vi "TMS Robot.vi"() -> ()   [LabVIEW 2018]
uses:
  <vilib>/Platform/TimedLoop/XDataNode/timing_clust.ctl
  <vilib>/Platform/TimedLoop/XDataNode/nitl_modes.ctl
  <vilib>/Platform/TimedLoop/XDataNode/wakeup.ctl
  <vilib>/myRIO/Instrument Drivers/Onboard IO/AI/typedefs/AI Reference.ctl
  <vilib>/myRIO/Common/Instrument Driver Framework/Utilities/typedefs/myRIO Generic Hardware Reference.ctl
  <vilib>/myRIO/Common/Instrument Driver Framework/Utilities/typedefs/Hardware Version Enum.ctl
  <vilib>/myRIO/Common/Instrument Driver Framework/Utilities/typedefs/myRIO v1.0 Reference.ctl
  <vilib>/myRIO/Common/Instrument Driver Framework/Utilities/typedefs/Generic FPGA Reference.ctl
  <vilib>/myRIO/Common/Instrument Driver Framework/myRIO v1.0/AI/typedefs/AI Channels List.ctl
  <vilib>/myRIO/Common/Instrument Driver Framework/myRIO v1.0/AI/typedefs/AI Channels Enum.ctl
  <vilib>/myRIO/Common/Instrument Driver Framework/Utilities/typedefs/Analog Scaling Constants List.ctl
  <vilib>/myRIO/Common/Instrument Driver Framework/Utilities/typedefs/Analog Scaling Constants.ctl
  <vilib>/userdefined/High Color/nirio_resource_hc.ctl
  <vilib>/myRIO/Instrument Drivers/Onboard IO/DIO/typedefs/DIO Reference.ctl
  <vilib>/myRIO/Common/Instrument Driver Framework/myRIO v1.0/DIO/typedefs/DIO Channels List.ctl
  <vilib>/myRIO/Common/Instrument Driver Framework/myRIO v1.0/DIO/typedefs/DIO Channels Enum.ctl
  <vilib>/myRIO/Common/Instrument Driver Framework/myRIO v1.0/AI/vis/myRIO v1.1 Open AI.vi
  <vilib>/myRIO/Common/Instrument Driver Framework/myRIO v1.0/DIO/vis/myRIO v1.1 Open DIO.vi
  <vilib>/myRIO/Common/Instrument Driver Framework/Utilities/vis/Validate Channels.vi
  <vilib>/myRIO/Common/Instrument Driver Framework/myRIO v1.0/AI/vis/myRIO v1.0 Reserve AI.vi
  <vilib>/myRIO/Common/Instrument Driver Framework/myRIO v1.0/DIO/vis/myRIO v1.0 Reserve DIO.vi
  <vilib>/myRIO/Common/Instrument Driver Framework/myRIO v1.0/DIO/vis/myRIO v1.0 Close DIO.vi
  <vilib>/myRIO/Common/Instrument Driver Framework/myRIO v1.0/AI/vis/myRIO v1.0 Build MUX Configuration AI.vi
  <vilib>/myRIO/Common/Instrument Driver Framework/myRIO v1.0/Resource Manager/vis/myRIO v1.0 Reserve Channel List.vi
  <vilib>/myRIO/Common/Instrument Driver Framework/myRIO v1.0/DIO/vis/myRIO v1.0 Build MUX Configuration DIO.vi
  <vilib>/myRIO/Common/Instrument Driver Framework/myRIO v1.0/DIO/vis/myRIO v1.0 Unreserve DIO.vi
  <vilib>/myRIO/Common/Instrument Driver Framework/myRIO v1.0/Resource Manager/vis/myRIO v1.0 Reserve Channel.vi
  <vilib>/myRIO/Common/Instrument Driver Framework/myRIO v1.0/Resource Manager/vis/myRIO v1.0 Unreserve Channel.vi
  <vilib>/myRIO/Common/Instrument Driver Framework/myRIO v1.0/Resource Manager/vis/myRIO v1.0 Create Configuration List.vi
  <vilib>/myRIO/Common/Instrument Driver Framework/myRIO v1.0/Resource Manager/vis/myRIO v1.0 Unreserve Channel List.vi
  <vilib>/myRIO/Common/Instrument Driver Framework/myRIO v1.0/Resource Manager/vis/myRIO v1.0 Build Mutex Name.vi
  <vilib>/Utility/VariantDataType/GetNumericInfo.vi
  <vilib>/Utility/error.llb/Error Cluster From Error Code.vi
  <vilib>/myRIO/Common/Instrument Driver Framework/myRIO v1.0/myRIO v1.1 Open.vi
  <vilib>/myRIO/Common/Instrument Driver Framework/Utilities/vis/IO Manager.vi
  <vilib>/myRIO/Common/Instrument Driver Framework/Utilities/vis/Configuration Manager.vi
  <vilib>/myRIO/Common/Instrument Driver Framework/myRIO v1.0/Resource Manager/vis/myRIO v1.0 Configure IO.vi
  <vilib>/myRIO/Common/Instrument Driver Framework/myRIO v1.0/myRIO v1.0 Close.vi
  <vilib>/myRIO/Common/Instrument Driver Framework/myRIO v1.0/AI/vis/myRIO v1.0 Get Scaling Constants AI.vi
  <vilib>/myRIO/Common/Instrument Driver Framework/myRIO v1.0/AI/vis/myRIO v1.0 Read AI.vi
  <vilib>/myRIO/Common/Instrument Driver Framework/myRIO v1.0/DIO/vis/myRIO v1.0 Write DIO.vi
  <vilib>/myRIO/Common/Instrument Driver Framework/myRIO v1.0/DIO/vis/myRIO v1.0 Shutdown DIO.vi
  <vilib>/platform/TimedLoop/XDataNode/XDataNode.xnode
  <vilib>/myRIO/Instrument Drivers/Onboard IO/DIO/vis/myRIO DIO Open.xnode
  <vilib>/myRIO/Instrument Drivers/Onboard IO/AI/vis/myRIO AI Open.xnode
  <vilib>/Platform/TimedLoop/XDataNode/XDNodeRunTimeDep.lvlib
  <vilib>/myRIO/Instrument Drivers/Onboard IO/DIO/DIO.lvlib
  <vilib>/myRIO/Instrument Drivers/Onboard IO/AI/AI.lvlib
panel:
  in  "Stop number L":dbl
  in  "Stop number R":dbl
  in  "Stop number x":dbl
  in  "Stop number y":dbl
  in  "Stop number z":dbl
  in  "Stop number psi":dbl
  out "up L":bool
  out "left L":bool
  in  "Step/s  curve":dbl=4.0
  in  "Step difference L":dbl
  in  "Tab Control":enum32{"Azimuth", "Elevation"}(tab)
  in  "Right":bool
  in  "Left":bool
  out "Real Output theta":dbl
  in  "User Input theta":dbl min=-45.0 max=45.0
  in  "Up":bool
  in  "Down":bool
  out "Real Output Phi":dbl
  in  "User Input Phi":dbl=10.45218049 min=9.2427 max=53.19163884
  in  "Motor Input L":dbl
  out "down L":bool
  out "right L":bool
  out "Moving":bool
  out "up R":bool
  out "left R":bool
  in  "Step difference R":dbl
  in  "Motor Input R":dbl
  out "down R":bool
  out "right R":bool
  out "Moving R":bool
  out "up z":bool
  out "down z":bool
  out "right z":bool
  out "left z":bool
  in  "Step/s z":dbl=4.0
  out "Motor Position z":dbl
  in  "User Input z":dbl min=-25.0 max=25.0
  out "Motor State z":dbl
  out "Real Output z":dbl
  in  "Step diff z":dbl
  in  "Up z":bool
  in  "Motor Input z":dbl
  in  "Down z":bool
  out "Moving z":bool
  out "up x":bool
  out "down x":bool
  out "right x":bool
  out "left x":bool
  in  "Step/s x":dbl=4.0
  out "Motor Position x":dbl
  in  "User Input x":dbl min=-25.0 max=25.0
  out "Motor State x":dbl
  out "Real Output x":dbl
  in  "Step diff x":dbl
  in  "Forward x":bool
  in  "Motor Input x":dbl
  in  "Backward x":bool
  out "Moving x":bool
  out "up y":bool
  out "down y":bool
  out "right y":bool
  out "left y":bool
  in  "Step/s y":dbl=4.0
  out "Motor Position y":dbl
  in  "User Input y":dbl min=-25.0 max=25.0
  out "Motor State y":dbl
  out "Real Output y":dbl
  in  "Step diff y":dbl
  in  "Left y":bool
  in  "Motor Input y":dbl
  in  "Right y":bool
  out "Moving y":bool
  out "up psi":bool
  out "down psi":bool
  out "right psi":bool
  out "left psi":bool
  in  "Step/s psi":dbl=4.0
  out "Motor Position psi":dbl
  in  "User Input psi":dbl min=-90.0 max=90.0
  out "Motor State psi":dbl
  out "Real Output psi":dbl
  in  "Step diff psi":dbl
  in  "Left psi":bool
  in  "Motor Input psi":dbl
  in  "Right psi":bool
  out "Moving psi":bool
  out "Homing x":bool
  out "Homing y":bool
  out "Homing z":bool
  out "Homing":bool
  out "Homing psi":bool
  in  "Stop":bool
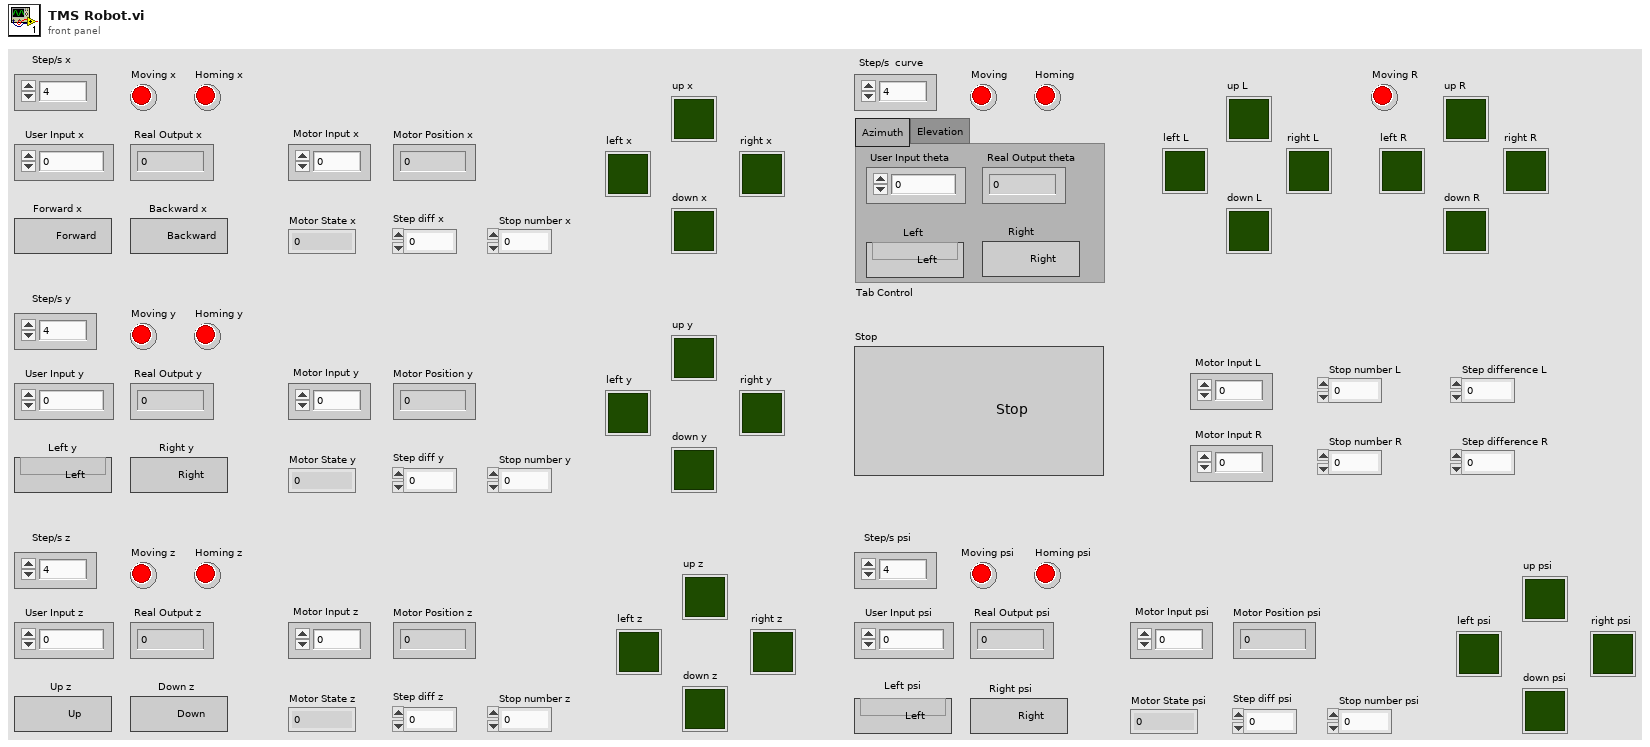
[diagram p1: front panel]
types:
  T1 = typedef "nirio_resource_hc.ctl" = tag
  T2 = typedef "Hardware Version Enum.ctl" = enum16{"Unknown", "myRIO-1900", "myRIO-1950", "roboRIO", "NI ELVIS RIO CM", "ELVIS III"}
  T3 = typedef "XDNodeRunTimeDep.lvlib/timing_clust.ctl" = cluster{"Expected End [f-1]":u64, "Actual End [f-1]":u64, "Finished Late? [f-1]":bool, "Expected End [i-1]":u64, "Actual End [i-1]":u64, "Finished Late? [i-1]":bool, "Expected Start [i]":u64, "Actual Start [i]":u64, "Expected Start [f]":u64, "Actual Start [f]":u64, "Source Name":string, "Structure Name":string, "Period":i64, "Deadline":i64, "Offset":i64, "Start":i64, "Priority":i32, "Timeout":i32, "Mode":T4, "Wakeup Reason":T5, "Error":errorcluster, "Source Type":string, "Secondary Source Type":string, "Global End Time":u64, "Global Start Time":u64, "Frame Duration":u64, "Iteration Duration":u64, "Assigned CPU":i32, "I/O Scan Engine Mode":u32}
  T4 = typedef "XDNodeRunTimeDep.lvlib/nitl_modes.ctl" = enum32{"No Change", "Process missed periods, maintain original phase", "Discard missed periods, maintain original phase", "Process missed periods, ignore original phase", "Discard missed periods, ignore original phase"}
  T5 = typedef "XDNodeRunTimeDep.lvlib/wakeup.ctl" = enum32{"Normal", "Aborted", "Asynchronous wakeup", "Timing source error", "Timed loop error", "Timeout"}
  T6 = typedef "AI.lvlib/AI Reference.ctl" = cluster{"myRIO Reference":T7, "AI Channels List":T10, "AI Scaling Constants List":T12}
  T7 = typedef "myRIO Generic Hardware Reference.ctl" = cluster{"myRIO Model":T2, "myRIO Hardware Reference":T8}
  T8 = typedef "myRIO v1.0 Reference.ctl" = cluster{"Generic FPGA Reference":T9, "Allow multiple opens":bool}
  T9 = typedef "Generic FPGA Reference.ctl" = refnum<k20>
  T10 = typedef "AI Channels List.ctl" = T11[]
  T11 = typedef "AI Channels Enum.ctl" = enum16{"Not Connected", "AudioIn/Left", "AudioIn/Right", "C/AI0", "C/AI1", "A/AI0", "A/AI1", "A/AI2", "A/AI3", "A/AI4", "A/AI5", "A/AI6", "A/AI7", "B/AI0", "B/AI1", "B/AI2", "B/AI3", "B/AI4", "B/AI5", "B/AI6", "B/AI7", "AI/AI0", "AI/AI1", "AI/AI2", "AI/AI3", "A/AI0 (DIFF)", "A/AI1 (DIFF)", "A/AI2 (DIFF)", "A/AI3 (DIFF)", "B/AI0 (DIFF)", "B/AI1 (DIFF)", "B/AI2 (DIFF)", "B/AI3 (DIFF)"}
  T12 = typedef "Analog Scaling Constants List.ctl" = T13[]
  T13 = typedef "Analog Scaling Constants.ctl" = cluster{"LSB Weight (Volts)":dbl, "Offset (Volts)":dbl, "Signed?":bool}
  T14 = typedef "DIO.lvlib/DIO Reference.ctl" = cluster{"myRIO Reference":T7, "DIO Channels List":T15}
  T15 = typedef "DIO Channels List.ctl" = T16[]
  T16 = typedef "DIO Channels Enum.ctl" = enum16{"Not Connected", "C/DIO0", "C/DIO1", "C/DIO2", "C/DIO3", "C/DIO4", "C/DIO5", "C/DIO6", "C/DIO7", "A/DIO0", "A/DIO1", "A/DIO2", "A/DIO3", "A/DIO4", "A/DIO5", "A/DIO6", "A/DIO7", "A/DIO8", "A/DIO9", "A/DIO10", "A/DIO11", "A/DIO12", "A/DIO13", "A/DIO14", "A/DIO15", "A/DIO16", "A/DIO17", "A/DIO18", "A/DIO19", "B/DIO0", "B/DIO1", "B/DIO2", "B/DIO3", "B/DIO4", "B/DIO5", "B/DIO6", "B/DIO7", "B/DIO8", "B/DIO9", "B/DIO10", "B/DIO11", "B/DIO12", "B/DIO13", "B/DIO14", "B/DIO15", "B/DIO16", "B/DIO17", "B/DIO18", "B/DIO19", "LED0", "LED1", "LED2", "LED3", "Button0", "DIO/DIO0", "DIO/DIO1", "DIO/DIO2", "DIO/DIO3", "DIO/DIO4", "DIO/DIO5", "DIO/DIO6", "DIO/DIO7", "DIO/DIO8", "DIO/DIO9", "SPI/CS0", "SPI/CS1", "SPI/CS2", "SPI/CS3", "LED RADIO (Green)", "LED RADIO (Red)", "LED COMM (Green)", "LED COMM (Red)", "LED MODE (Green)", "LED MODE (Red)"}
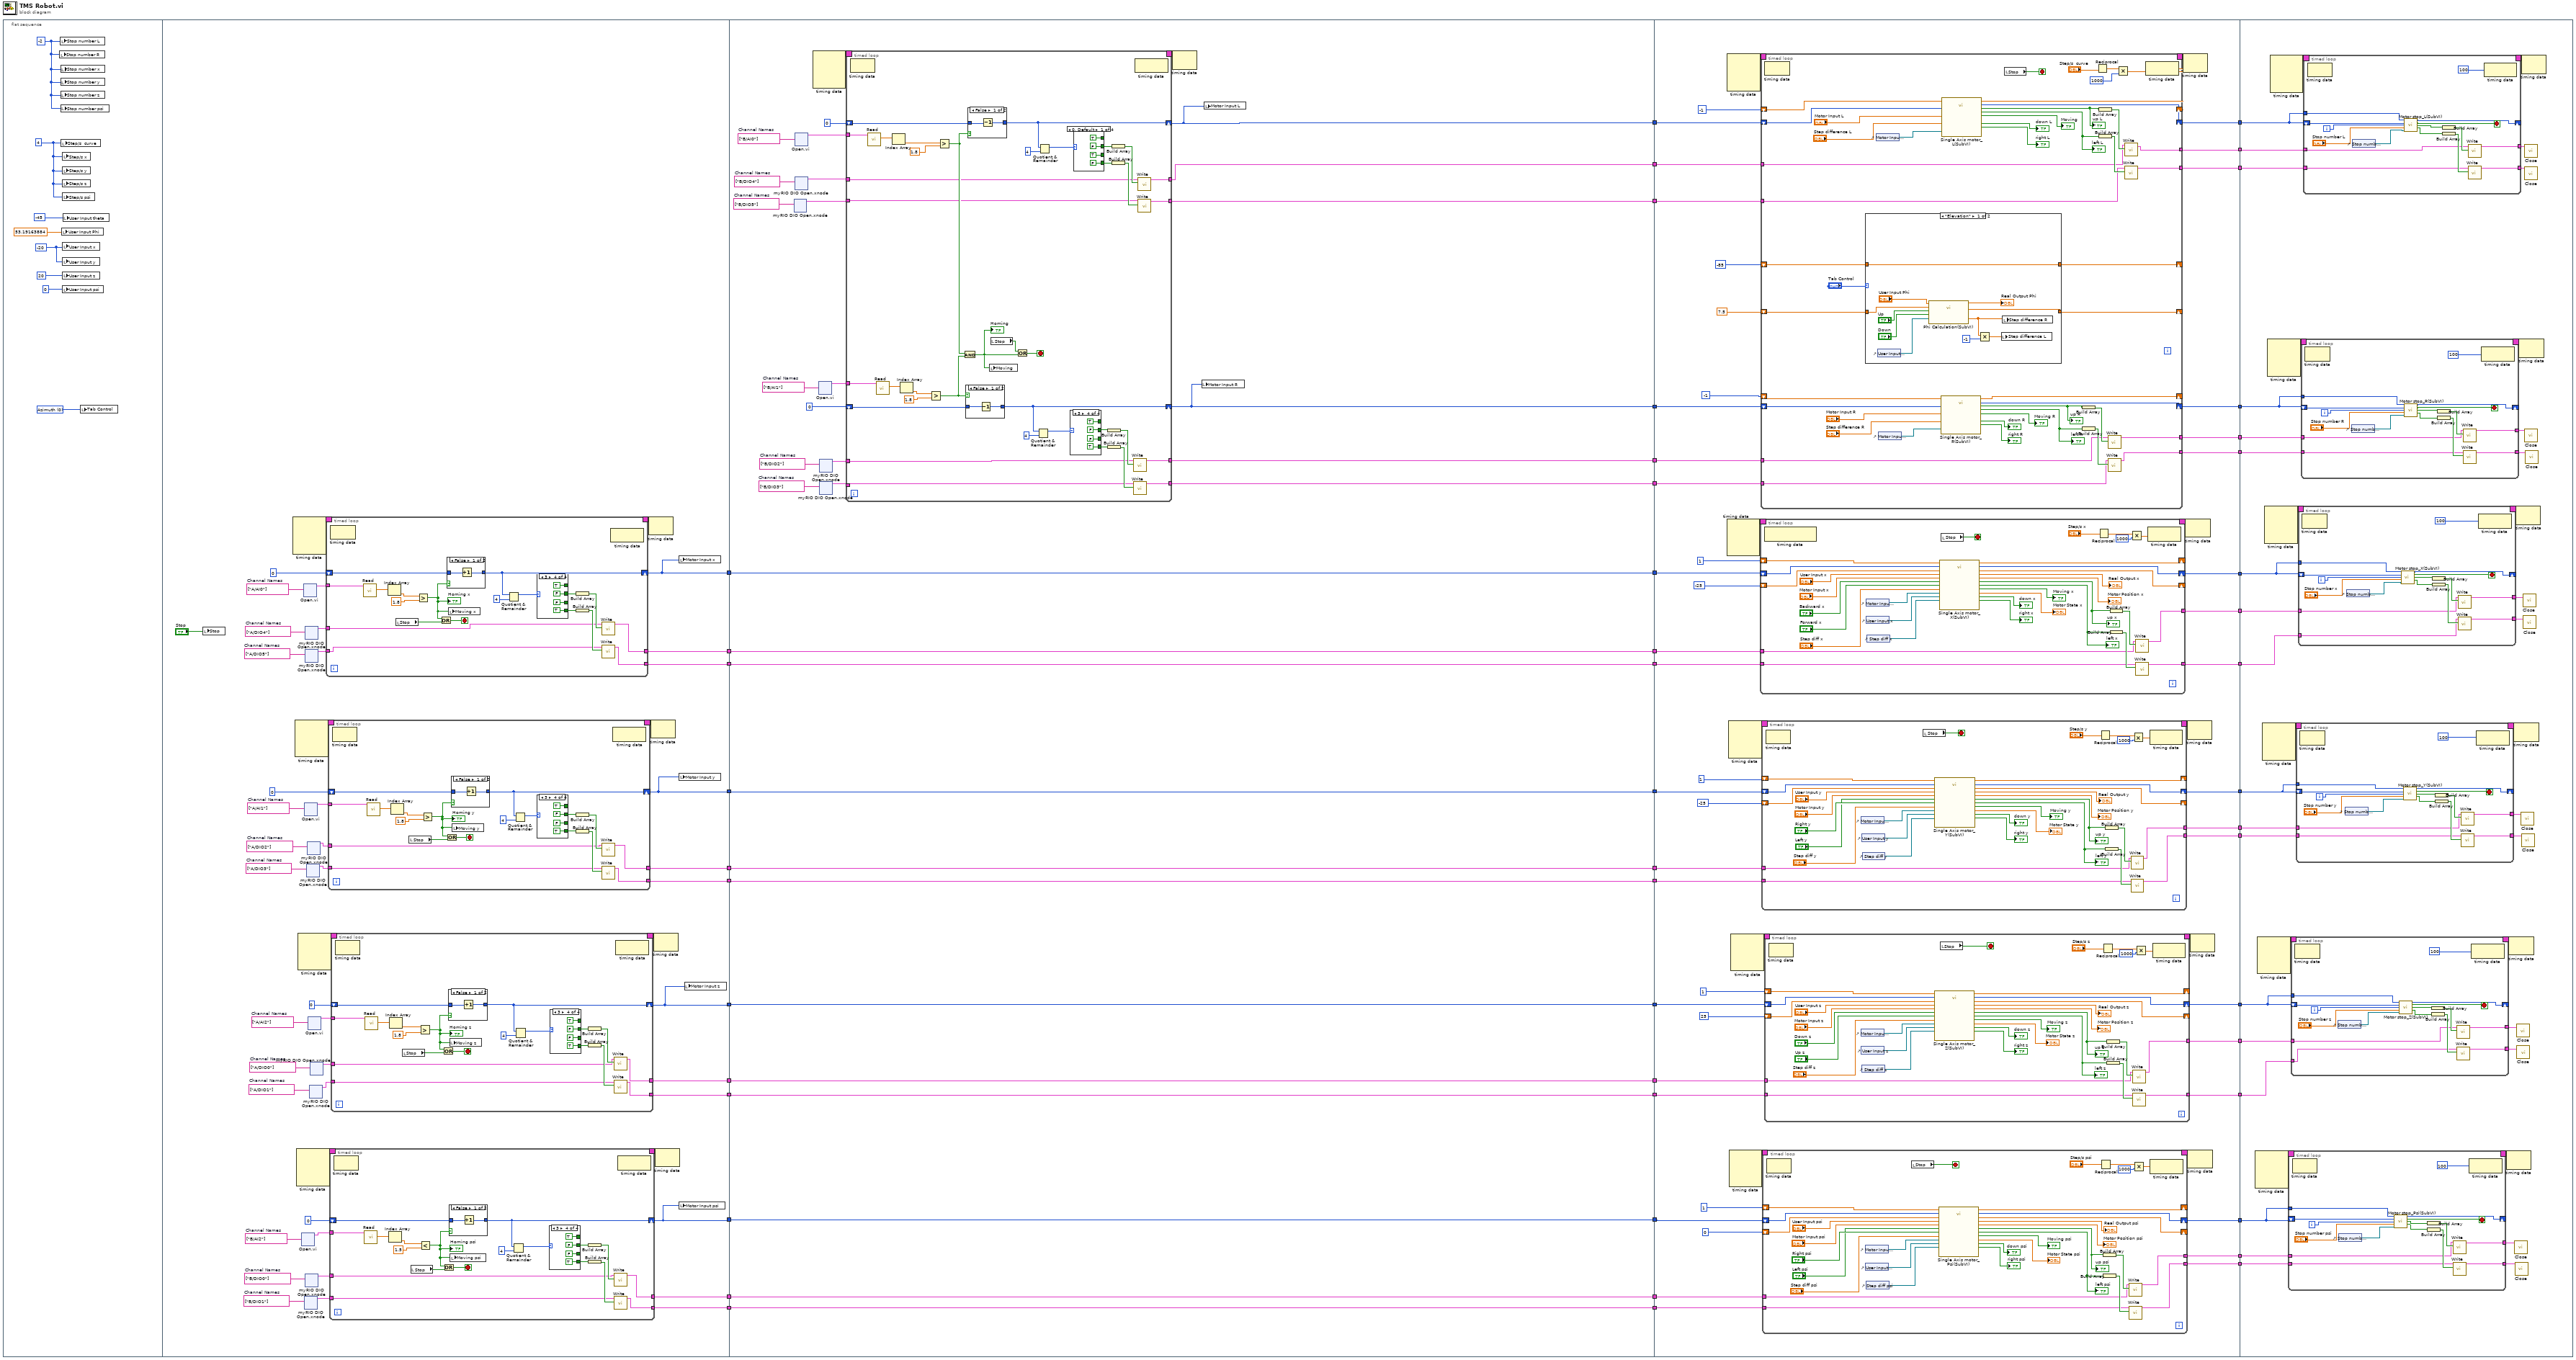
[diagram p0: block diagram]
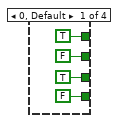
[diagram p2: hidden frame]
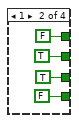
[diagram p3: hidden frame]
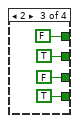
[diagram p4: hidden frame]
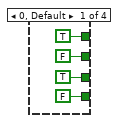
[diagram p6: hidden frame]
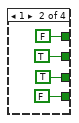
[diagram p7: hidden frame]
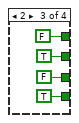
[diagram p8: hidden frame]
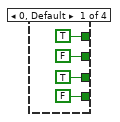
[diagram p10: hidden frame]
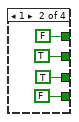
[diagram p11: hidden frame]
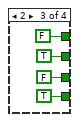
[diagram p12: hidden frame]
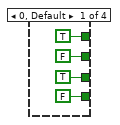
[diagram p15: hidden frame]
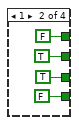
[diagram p16: hidden frame]
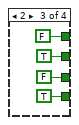
[diagram p17: hidden frame]
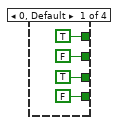
[diagram p18: hidden frame]
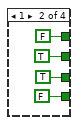
[diagram p19: hidden frame]
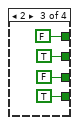
[diagram p20: hidden frame]
diagram:
  n1 = flat-sequence {
    tunnel: [w92] -> w30
    tunnel: [w91] -> w28
    tunnel: [w93] -> w26
    tunnel: [w90] -> w24
    tunnel: [w72] -> w22
    tunnel: [w71] -> w20
    tunnel: [w70] -> w18
    tunnel: [w69] -> w16
    tunnel: [w68] -> w14
    tunnel: [w67] -> w12
    tunnel: [w66] -> w10
    tunnel: [w65] -> w8
    tunnel: w30 -> [w507]
    tunnel: [w507] -> w29
    tunnel: w28 -> [w506]
    tunnel: [w506] -> w27
    tunnel: w26 -> [w505]
    tunnel: [w505] -> w25
    tunnel: w24 -> [w504]
    tunnel: [w504] -> w23
    tunnel: w22 -> [w503]
    tunnel: [w503] -> w21
    tunnel: w20 -> [w502]
    tunnel: [w502] -> w19
    tunnel: w18 -> [w501]
    tunnel: [w501] -> w17
    tunnel: w16 -> [w500]
    tunnel: [w500] -> w15
    tunnel: w14 -> [w499]
    tunnel: [w499] -> w13
    tunnel: w12 -> [w498]
    tunnel: [w498] -> w11
    tunnel: w10 -> [w497]
    tunnel: [w497] -> w9
    tunnel: w8 -> [w496]
    tunnel: [w496] -> w7
    tunnel: [w485] -> w6
    tunnel: [w484] -> w5
    tunnel: [w483] -> w4
    tunnel: [w482] -> w3
    tunnel: [w481] -> w2
    tunnel: [w480] -> w1
    tunnel: w29 -> [w723]
    tunnel: w27 -> [w722]
    tunnel: w25 -> [w721]
    tunnel: w23 -> [w719]
    tunnel: [w717] -> w48
    tunnel: [w716] -> w47
    tunnel: [w715] -> w46
    tunnel: [w714] -> w45
    tunnel: [w713] -> w44
    tunnel: [w712] -> w43
    tunnel: w21 -> [w710]
    tunnel: w19 -> [w709]
    tunnel: w17 -> [w708]
    tunnel: w15 -> [w707]
    tunnel: w13 -> [w706]
    tunnel: w11 -> [w705]
    tunnel: w9 -> [w704]
    tunnel: w7 -> [w703]
    tunnel: [w698] -> w42
    tunnel: [w697] -> w41
    tunnel: [w696] -> w40
    tunnel: [w695] -> w39
    tunnel: [w694] -> w38
    tunnel: [w693] -> w37
    tunnel: [w692] -> w36
    tunnel: [w691] -> w35
    tunnel: [w690] -> w34
    tunnel: [w689] -> w33
    tunnel: [w688] -> w32
    tunnel: [w687] -> w31
    tunnel: w6 -> [w701]
    tunnel: w5 -> [w702]
    tunnel: w4 -> [w711]
    tunnel: w3 -> [w700]
    tunnel: w2 -> [w699]
    tunnel: w1 -> [w720]
    tunnel: w48 -> [w1012]
    tunnel: w47 -> [w1009]
    tunnel: w46 -> [w1006]
    tunnel: w45 -> [w1003]
    tunnel: w44 -> [w1000]
    tunnel: w43 -> [w997]
    tunnel: w42 -> [w994]
    tunnel: w41 -> [w993]
    tunnel: w40 -> [w992]
    tunnel: w39 -> [w991]
    tunnel: w38 -> [w986]
    tunnel: w37 -> [w985]
    tunnel: w36 -> [w984]
    tunnel: w35 -> [w983]
    tunnel: w34 -> [w982]
    tunnel: w33 -> [w981]
    tunnel: w32 -> [w980]
    tunnel: w31 -> [w979]
    frame #0 {
      w49 = u16 0 items=["Azimuth"]
      w51 = -20
      w55 = -2
      w54 = 4
      n2 = local write "Stop number R"(w55) -> ()
      n3 = local write "Stop number L"(w55) -> ()
      n4 = local write "Stop number x"(w55) -> ()
      n5 = local write "Stop number y"(w55) -> ()
      n6 = local write "Stop number z"(w55) -> ()
      n7 = local write "Stop number psi"(w55) -> ()
      n8 = local write "Step/s  curve"(w54) -> ()
      n9 = local write "User Input Phi"(53.19163884) -> ()
      n10 = local write "Step/s x"(w54) -> ()
      n11 = local write "Step/s y"(w54) -> ()
      n12 = local write "Step/s z"(w54) -> ()
      n13 = local write "Step/s psi"(w54) -> ()
      n14 = local write "User Input x"(w51) -> ()
      n15 = local write "User Input y"(w51) -> ()
      n16 = local write "User Input z"(20) -> ()
      n17 = local write "User Input psi"(0) -> ()
      n18 = local write "User Input theta"(-45) -> ()
      n19 = local write "Tab Control"(w49) -> ()
    }
    frame #1 {
      w58 = tag[] ["B/AI2"]  # Channel Names
      w60 = tag[] ["A/AI2"]  # Channel Names
      w62 = tag[] ["A/AI1"]  # Channel Names
      w64 = tag[] ["A/AI0"]  # Channel Names
      w76 = tag[] ["B/DIO1"]  # Channel Names
      w75 = tag[] ["B/DIO0"]  # Channel Names
      w80 = tag[] ["A/DIO1"]  # Channel Names
      w79 = tag[] ["A/DIO0"]  # Channel Names
      w84 = tag[] ["A/DIO3"]  # Channel Names
      w83 = tag[] ["A/DIO2"]  # Channel Names
      w88 = tag[] ["A/DIO5"]  # Channel Names
      w87 = tag[] ["A/DIO4"]  # Channel Names
      n20 = local write "Stop"("Stop") -> ()
      n21 = node-c288() -> (w105:T3)  [unwired: 4 in]
      n22 = node-c288() -> (w102:T3)  [unwired: 4 in]
      n23 = node-c288() -> (w96:T3)  [unwired: 4 in]
      n24 = node-c288() -> (w99:T3)  [unwired: 4 in]
      n25 = xnode "Open.vi"("Channel Names"=w58) -> ("AI Ref Out"=w57:T6)  [unwired: 2 in, 1 out]
      n26 = xnode "Open.vi"("Channel Names"=w64) -> ("AI Ref Out"=w63:T6)  [unwired: 2 in, 1 out]
      n27 = xnode "Open.vi"("Channel Names"=w62) -> ("AI Ref Out"=w61:T6)  [unwired: 2 in, 1 out]
      n28 = xnode "myRIO DIO Open.xnode"("Channel Names"=w76) -> ("DIO Ref Out"=w73:T14)  [unwired: 2 in, 1 out]
      n29 = xnode "myRIO DIO Open.xnode"("Channel Names"=w88) -> ("DIO Ref Out"=w85:T14)  [unwired: 2 in, 1 out]
      n30 = xnode "myRIO DIO Open.xnode"("Channel Names"=w75) -> ("DIO Ref Out"=w74:T14)  [unwired: 2 in, 1 out]
      n31 = xnode "myRIO DIO Open.xnode"("Channel Names"=w87) -> ("DIO Ref Out"=w86:T14)  [unwired: 2 in, 1 out]
      n32 = xnode "myRIO DIO Open.xnode"("Channel Names"=w84) -> ("DIO Ref Out"=w81:T14)  [unwired: 2 in, 1 out]
      n33 = xnode "myRIO DIO Open.xnode"("Channel Names"=w83) -> ("DIO Ref Out"=w82:T14)  [unwired: 2 in, 1 out]
      n34 = xnode "Open.vi"("Channel Names"=w60) -> ("AI Ref Out"=w59:T6)  [unwired: 2 in, 1 out]
      n35 = xnode "myRIO DIO Open.xnode"("Channel Names"=w80) -> ("DIO Ref Out"=w77:T14)  [unwired: 2 in, 1 out]
      n36 = xnode "myRIO DIO Open.xnode"("Channel Names"=w79) -> ("DIO Ref Out"=w78:T14)  [unwired: 2 in, 1 out]
      n37 = timed-loop {
        timing: w105 -> [_]
        timing-out: [_] -> w104
        shift-right: [w446] -> w92
        shift-left: 0 -> [w447]
        tunnel: w86 -> [w438]
        tunnel: w85 -> [w437]
        tunnel: [w436] -> w66
        tunnel: [w435] -> w65
        tunnel: w63 -> [w432]
        stop <- w444 stop-if-true
        n38 = node-c288() -> ()  [unwired: 1 in, 1 out]
        n39 = call <vilib>:"Read.vi"("AI Ref In"=w432) -> ("Values"=w434:dbl[])  [unwired: 8 in, 2 out]
        n40 = Index Array(array=w434) -> (element=w433:dbl)  [unwired: 1 in]
        n41 = local read "Stop"() -> (w445:bool)
        n42 = Greater?(x=w433, y=1.8) -> (0:w443:bool)
        "Homing x" <- w443
        n43 = Or(x=w443, y=w445) -> (x .or. y?=w444:bool)
        n44 = case shown="False" w443 {
          tunnel: w447 -> [w452 w453]
          tunnel: [w451 w453] -> w446
          frame False {
            n45 = Increment(x=w452) -> (x+1=w451:i32)
          }
          frame True {
          }
        }
        n46 = local write "Moving x"(w443) -> ()
        n47 = Quotient & Remainder(x=w446, y=4) -> (x-y*floor(x/y)=w449:i32)  [unwired: 1 out]
        n48 = case shown="3" w449 {
          tunnel: [FALSE FALSE TRUE TRUE] -> w439
          tunnel: [TRUE TRUE FALSE FALSE] -> _
          tunnel: [FALSE TRUE TRUE FALSE] -> w440
          tunnel: [TRUE FALSE FALSE TRUE] -> _
          frame 0, Default {
          }
          frame 1 {
          }
          frame 2 {
          }
          frame 3 {
          }
        }
        n49 = Build Array(w440) -> (w442:bool[])
        n50 = Build Array(w439) -> (w441:bool[])
        n51 = call <vilib>:"Write.vi"("Values"=w442, "DIO Ref In"=w438) -> ("DIO Ref Out"=w436:T14)  [unwired: 7 in, 1 out]
        n52 = call <vilib>:"Write.vi"("Values"=w441, "DIO Ref In"=w437) -> ("DIO Ref Out"=w435:T14)  [unwired: 7 in, 1 out]
        n53 = node-c288() -> ()  [unwired: 1 in, 1 out]
      }
      n54 = timed-loop {
        timing: w102 -> [_]
        timing-out: [_] -> w101
        shift-right: [w405] -> w91
        shift-left: 0 -> [w406]
        tunnel: w82 -> [w396]
        tunnel: w81 -> [w395]
        tunnel: [w394] -> w68
        tunnel: [w393] -> w67
        tunnel: w61 -> [w390]
        stop <- w402 stop-if-true
        n55 = node-c288() -> ()  [unwired: 1 in, 1 out]
        n56 = call <vilib>:"Read.vi"("AI Ref In"=w390) -> ("Values"=w392:dbl[])  [unwired: 8 in, 2 out]
        n57 = Index Array(array=w392) -> (element=w391:dbl)  [unwired: 1 in]
        n58 = local read "Stop"() -> (w403:bool)
        n59 = Greater?(x=w391, y=1.8) -> (0:w401:bool)
        "Homing y" <- w401
        n60 = Or(x=w401, y=w403) -> (x .or. y?=w402:bool)
        n61 = case shown="False" w401 {
          tunnel: w406 -> [w426 w427]
          tunnel: [w425 w427] -> w405
          frame False {
            n62 = Increment(x=w426) -> (x+1=w425:i32)
          }
          frame True {
          }
        }
        n63 = local write "Moving y"(w401) -> ()
        n64 = Quotient & Remainder(x=w405, y=4) -> (x-y*floor(x/y)=w404:i32)  [unwired: 1 out]
        n65 = case shown="3" w404 {
          tunnel: [FALSE FALSE TRUE TRUE] -> w397
          tunnel: [TRUE TRUE FALSE FALSE] -> _
          tunnel: [FALSE TRUE TRUE FALSE] -> w398
          tunnel: [TRUE FALSE FALSE TRUE] -> _
          frame 0, Default {
          }
          frame 1 {
          }
          frame 2 {
          }
          frame 3 {
          }
        }
        n66 = Build Array(w398) -> (w400:bool[])
        n67 = Build Array(w397) -> (w399:bool[])
        n68 = call <vilib>:"Write.vi"("Values"=w400, "DIO Ref In"=w396) -> ("DIO Ref Out"=w394:T14)  [unwired: 7 in, 1 out]
        n69 = call <vilib>:"Write.vi"("Values"=w399, "DIO Ref In"=w395) -> ("DIO Ref Out"=w393:T14)  [unwired: 7 in, 1 out]
        n70 = node-c288() -> ()  [unwired: 1 in, 1 out]
      }
      n71 = timed-loop {
        timing: w96 -> [_]
        timing-out: [_] -> w95
        shift-right: [w321] -> w90
        shift-left: 0 -> [w322]
        tunnel: w74 -> [w312]
        tunnel: w73 -> [w311]
        tunnel: [w310] -> w70
        tunnel: [w309] -> w69
        tunnel: w57 -> [w306]
        stop <- w318 stop-if-true
        n72 = node-c288() -> ()  [unwired: 1 in, 1 out]
        n73 = call <vilib>:"Read.vi"("AI Ref In"=w306) -> ("Values"=w308:dbl[])  [unwired: 8 in, 2 out]
        n74 = Index Array(array=w308) -> (element=w307:dbl)  [unwired: 1 in]
        n75 = local read "Stop"() -> (w319:bool)
        n76 = Less?(x=w307, y=1.5) -> (x < y?=w317:bool)
        "Homing psi" <- w317
        n77 = Or(x=w317, y=w319) -> (x .or. y?=w318:bool)
        n78 = case shown="False" w317 {
          tunnel: w322 -> [w342 w343]
          tunnel: [w341 w343] -> w321
          frame False {
            n79 = Increment(x=w342) -> (x+1=w341:i32)
          }
          frame True {
          }
        }
        n80 = local write "Moving psi"(w317) -> ()
        n81 = Quotient & Remainder(x=w321, y=4) -> (x-y*floor(x/y)=w320:i32)  [unwired: 1 out]
        n82 = case shown="3" w320 {
          tunnel: [FALSE FALSE TRUE TRUE] -> w313
          tunnel: [TRUE TRUE FALSE FALSE] -> _
          tunnel: [FALSE TRUE TRUE FALSE] -> w314
          tunnel: [TRUE FALSE FALSE TRUE] -> _
          frame 0, Default {
          }
          frame 1 {
          }
          frame 2 {
          }
          frame 3 {
          }
        }
        n83 = Build Array(w314) -> (w316:bool[])
        n84 = Build Array(w313) -> (w315:bool[])
        n85 = call <vilib>:"Write.vi"("Values"=w316, "DIO Ref In"=w312) -> ("DIO Ref Out"=w310:T14)  [unwired: 7 in, 1 out]
        n86 = call <vilib>:"Write.vi"("Values"=w315, "DIO Ref In"=w311) -> ("DIO Ref Out"=w309:T14)  [unwired: 7 in, 1 out]
        n87 = node-c288() -> ()  [unwired: 1 in, 1 out]
      }
      n88 = timed-loop {
        timing: w99 -> [_]
        timing-out: [_] -> w98
        shift-right: [w363] -> w93
        shift-left: 0 -> [w364]
        tunnel: w78 -> [w354]
        tunnel: w77 -> [w353]
        tunnel: [w352] -> w72
        tunnel: [w351] -> w71
        tunnel: w59 -> [w348]
        stop <- w360 stop-if-true
        n89 = node-c288() -> ()  [unwired: 1 in, 1 out]
        n90 = call <vilib>:"Read.vi"("AI Ref In"=w348) -> ("Values"=w350:dbl[])  [unwired: 8 in, 2 out]
        n91 = Index Array(array=w350) -> (element=w349:dbl)  [unwired: 1 in]
        n92 = local read "Stop"() -> (w361:bool)
        n93 = Greater?(x=w349, y=1.8) -> (0:w359:bool)
        "Homing z" <- w359
        n94 = Or(x=w359, y=w361) -> (x .or. y?=w360:bool)
        n95 = case shown="False" w359 {
          tunnel: w364 -> [w384 w385]
          tunnel: [w383 w385] -> w363
          frame False {
            n96 = Increment(x=w384) -> (x+1=w383:i32)
          }
          frame True {
          }
        }
        n97 = local write "Moving z"(w359) -> ()
        n98 = Quotient & Remainder(x=w363, y=4) -> (x-y*floor(x/y)=w362:i32)  [unwired: 1 out]
        n99 = case shown="3" w362 {
          tunnel: [FALSE FALSE TRUE TRUE] -> w355
          tunnel: [TRUE TRUE FALSE FALSE] -> _
          tunnel: [FALSE TRUE TRUE FALSE] -> w356
          tunnel: [TRUE FALSE FALSE TRUE] -> _
          frame 0, Default {
          }
          frame 1 {
          }
          frame 2 {
          }
          frame 3 {
          }
        }
        n100 = Build Array(w356) -> (w358:bool[])
        n101 = Build Array(w355) -> (w357:bool[])
        n102 = call <vilib>:"Write.vi"("Values"=w358, "DIO Ref In"=w354) -> ("DIO Ref Out"=w352:T14)  [unwired: 7 in, 1 out]
        n103 = call <vilib>:"Write.vi"("Values"=w357, "DIO Ref In"=w353) -> ("DIO Ref Out"=w351:T14)  [unwired: 7 in, 1 out]
        n104 = node-c288() -> ()  [unwired: 1 in, 1 out]
      }
      n105 = node-c288(w104) -> ()  [unwired: 1 out]
      n106 = node-c288(w101) -> ()  [unwired: 1 out]
      n107 = node-c288(w98) -> ()  [unwired: 1 out]
      n108 = node-c288(w95) -> ()  [unwired: 1 out]
      n109 = local write "Motor Input x"(w92) -> ()
      n110 = local write "Motor Input y"(w91) -> ()
      n111 = local write "Motor Input psi"(w90) -> ()
      n112 = local write "Motor Input z"(w93) -> ()
    }
    frame #2 {
      w476 = tag[] ["B/AI1"]  # Channel Names
      w479 = tag[] ["B/AI0"]  # Channel Names
      w474 = tag[] ["B/DIO3"]  # Channel Names
      w475 = tag[] ["B/DIO2"]  # Channel Names
      w477 = tag[] ["B/DIO5"]  # Channel Names
      w478 = tag[] ["B/DIO4"]  # Channel Names
      n113 = xnode "myRIO DIO Open.xnode"("Channel Names"=w477) -> ("DIO Ref Out"=w489:T14)  [unwired: 2 in, 1 out]
      n114 = xnode "Open.vi"("Channel Names"=w479) -> ("AI Ref Out"=w492:T6)  [unwired: 2 in, 1 out]
      n115 = xnode "myRIO DIO Open.xnode"("Channel Names"=w478) -> ("DIO Ref Out"=w488:T14)  [unwired: 2 in, 1 out]
      n116 = node-c288() -> (w495:T3)  [unwired: 4 in]
      n117 = xnode "Open.vi"("Channel Names"=w476) -> ("AI Ref Out"=w493:T6)  [unwired: 2 in, 1 out]
      n118 = xnode "myRIO DIO Open.xnode"("Channel Names"=w474) -> ("DIO Ref Out"=w491:T14)  [unwired: 2 in, 1 out]
      n119 = xnode "myRIO DIO Open.xnode"("Channel Names"=w475) -> ("DIO Ref Out"=w490:T14)  [unwired: 2 in, 1 out]
      n120 = timed-loop {
        timing: w495 -> [_]
        timing-out: [_] -> w494
        shift-right: [w641] -> w480
        shift-left: 0 -> [w642]
        shift-right: [w636] -> w483
        shift-left: 0 -> [w635]
        tunnel: [w625] -> w481
        tunnel: [w624] -> w482
        tunnel: w488 -> [w623]
        tunnel: w489 -> [w622]
        tunnel: w490 -> [w617]
        tunnel: w491 -> [w616]
        tunnel: [w615] -> w484
        tunnel: [w614] -> w485
        tunnel: w492 -> [w611]
        tunnel: w493 -> [w608]
        stop <- w634 stop-if-true
        n121 = node-c288() -> ()  [unwired: 1 in, 1 out]
        n122 = call <vilib>:"Read.vi"("AI Ref In"=w611) -> ("Values"=w613:dbl[])  [unwired: 8 in, 2 out]
        n123 = call <vilib>:"Read.vi"("AI Ref In"=w608) -> ("Values"=w610:dbl[])  [unwired: 8 in, 2 out]
        n124 = Index Array(array=w613) -> (element=w612:dbl)  [unwired: 1 in]
        n125 = Index Array(array=w610) -> (element=w609:dbl)  [unwired: 1 in]
        n126 = Greater?(x=w609, y=1.8) -> (0:w631:bool)
        n127 = Greater?(x=w612, y=1.8) -> (0:w633:bool)
        n128 = And(x=w633, y=w631) -> (x .and. y?=w630:bool)
        "Homing" <- w630
        n129 = case shown="False" w631 {
          tunnel: [w662 w663] -> w636
          tunnel: w635 -> [w661 w663]
          frame False {
            n130 = Decrement(x=w661) -> (x-1=w662:i32)
          }
          frame True {
          }
        }
        n131 = case shown="False" w633 {
          tunnel: w642 -> [w681 w682]
          tunnel: [w680 w682] -> w641
          frame False {
            n132 = Decrement(x=w681) -> (x-1=w680:i32)
          }
          frame True {
          }
        }
        n133 = local write "Moving"(w630) -> ()
        n134 = local read "Stop"() -> (w632:bool)
        n135 = Or(x=w632, y=w630) -> (x .or. y?=w634:bool)
        n136 = Quotient & Remainder(x=w636, y=4) -> (x-y*floor(x/y)=w637:i32)  [unwired: 1 out]
        n137 = Quotient & Remainder(x=w641, y=4) -> (x-y*floor(x/y)=w640:i32)  [unwired: 1 out]
        n138 = case shown="3" w637 {
          tunnel: [FALSE FALSE TRUE TRUE] -> w618
          tunnel: [TRUE TRUE FALSE FALSE] -> _
          tunnel: [FALSE TRUE TRUE FALSE] -> w619
          tunnel: [TRUE FALSE FALSE TRUE] -> _
          frame 0, Default {
          }
          frame 1 {
          }
          frame 2 {
          }
          frame 3 {
          }
        }
        n139 = case shown="0, Default" w640 {
          tunnel: [FALSE FALSE TRUE TRUE] -> w626
          tunnel: [TRUE TRUE FALSE FALSE] -> _
          tunnel: [FALSE TRUE TRUE FALSE] -> w627
          tunnel: [TRUE FALSE FALSE TRUE] -> _
          frame 0, Default {
          }
          frame 1 {
          }
          frame 2 {
          }
          frame 3 {
          }
        }
        n140 = Build Array(w619) -> (w621:bool[])
        n141 = Build Array(w618) -> (w620:bool[])
        n142 = Build Array(w627) -> (w629:bool[])
        n143 = Build Array(w626) -> (w628:bool[])
        n144 = call <vilib>:"Write.vi"("Values"=w621, "DIO Ref In"=w617) -> ("DIO Ref Out"=w615:T14)  [unwired: 7 in, 1 out]
        n145 = call <vilib>:"Write.vi"("Values"=w620, "DIO Ref In"=w616) -> ("DIO Ref Out"=w614:T14)  [unwired: 7 in, 1 out]
        n146 = node-c288() -> ()  [unwired: 1 in, 1 out]
        n147 = call <vilib>:"Write.vi"("Values"=w629, "DIO Ref In"=w623) -> ("DIO Ref Out"=w625:T14)  [unwired: 7 in, 1 out]
        n148 = call <vilib>:"Write.vi"("Values"=w628, "DIO Ref In"=w622) -> ("DIO Ref Out"=w624:T14)  [unwired: 7 in, 1 out]
      }
      n149 = node-c288(w494) -> ()  [unwired: 1 out]
      n150 = local write "Motor Input R"(w483) -> ()
      n151 = local write "Motor Input L"(w480) -> ()
    }
    frame #3 {
      n152 = node-c288() -> (w737:T3)  [unwired: 4 in]
      n153 = node-c288() -> (w744:T3)  [unwired: 4 in]
      n154 = node-c288() -> (w735:T3)  [unwired: 4 in]
      n155 = node-c288() -> (w727:T3)  [unwired: 4 in]
      n156 = node-c288() -> (w739:T3)  [unwired: 4 in]
      n157 = timed-loop {
        shift-right: [w839] -> w715
        shift-left: w723 -> [w850]
        shift-right: [w840] -> _
        shift-left: 1 -> [w851]
        shift-right: [w835] -> _
        shift-left: -25 -> [w849]
        timing: w737 -> [_]
        timing-out: [_] -> w736
        tunnel: w704 -> [w826]
        tunnel: w703 -> [w825]
        tunnel: [w824] -> w694
        tunnel: [w823] -> w693
        stop <- w833 stop-if-true
        n158 = node-c288() -> ()  [unwired: 1 in, 1 out]
        n159 = control-ref of="Motor Input x"() -> (w843:refnum<vi>)
        n160 = control-ref of="User Input x"() -> (w842:refnum<vi>)
        n161 = control-ref of="Step diff x"() -> (w841:refnum<vi>)
        n162 = call "Single Axis motor_X(SubVI).vi"("State=1, I"=w851, "Motor=0, I"=w850, "Position=0, I"=w849, "User Input"="User Input x", "Motor Input"="Motor Input x", "Backward"="Backward x", "Forward"="Forward x", "Step diff"="Step diff x", "Motor input_L"=w843, "User input_L"=w842, "Step diff_L"=w841) -> ("right"=→"right x":bool, "down"=→"down x":bool, "Motor State"=→"Motor State x":dbl, "State=1, O"=w840:dbl, "Motor=0, O"=w839:i32, "Position=0, O"=w835:dbl, "Real Output"=→"Real Output x":dbl, "Motor Position"=→"Motor Position x":dbl, "up"=w828:bool, "left"=w827:bool, "Moving"=→"Moving x":bool)  [unwired: 5 in, 1 out]
        "up x" <- w828
        "left x" <- w827
        n163 = local read "Stop"() -> (w833:bool)
        n164 = Reciprocal(x="Step/s x") -> (1/x=w854:dbl)
        n165 = Build Array(w828) -> (w830:bool[])
        n166 = Build Array(w827) -> (w829:bool[])
        n167 = Multiply(x=w854, y=1000) -> (x*y=w852:dbl)
        n168 = call <vilib>:"Write.vi"("Values"=w830, "DIO Ref In"=w826) -> ("DIO Ref Out"=w823:T14)  [unwired: 7 in, 1 out]
        n169 = call <vilib>:"Write.vi"("Values"=w829, "DIO Ref In"=w825) -> ("DIO Ref Out"=w824:T14)  [unwired: 7 in, 1 out]
        n170 = node-c288(w852) -> ()  [unwired: 1 out]
      }
      n171 = timed-loop {
        shift-right: [w934] -> w717
        shift-left: w720 -> [w935]
        shift-right: [w936] -> _
        shift-left: -1 -> [w937]
        shift-right: [w941] -> _
        shift-left: -85 -> [w942]
        timing: w744 -> [_]
        timing-out: [_] -> w743
        shift-right: [w939] -> _
        shift-left: 7.5 -> [w938]
        shift-right: [w923] -> w716
        shift-left: w711 -> [w924]
        shift-right: [w921] -> _
        shift-left: -1 -> [w922]
        tunnel: w702 -> [w912]
        tunnel: w701 -> [w911]
        tunnel: w700 -> [w906]
        tunnel: w699 -> [w905]
        tunnel: [w904] -> w698
        tunnel: [w903] -> w697
        tunnel: [w902] -> w696
        tunnel: [w901] -> w695
        stop <- w929 stop-if-true
        n172 = node-c288() -> ()  [unwired: 1 in, 1 out]
        n173 = case shown="\"Elevation\"" "Tab Control" {
          tunnel: w938 -> [w956 w966]
          tunnel: [w955 w966] -> w939
          tunnel: w942 -> [w957 w963]
          tunnel: [w957 w962] -> w941
          frame "Elevation" {
            n174 = control-ref of="User Input Phi"() -> (w950:refnum<vi>)
            n175 = call "Phi Calculation(SubVI).vi"(0:"User Input Phi"="User Input Phi", "Position=0, I"=w956, "Up"="Up", "Down"="Down", 11:"User Input Phi"=w950) -> ("Real output phi"=→"Real Output Phi":dbl, "Position=0, O"=w955:dbl, "Step diff"=w947:dbl)  [unwired: 8 in]
            n176 = Multiply(x=w947, y=-1) -> (x*y=w948:dbl)
            n177 = local write "Step difference L"(w948) -> ()
            n178 = local write "Step difference R"(w947) -> ()
          }
          frame "Azimuth" {
            n179 = control-ref of="User Input theta"() -> (w964:refnum<vi>)
            n180 = call "Theta Calculation(SubVI).vi"(0:"User Input theta"="User Input theta", "Position=-85, I"=w963, "Right"="Right", "Left"="Left", 11:"User Input theta"=w964) -> ("Position=-85, O"=w962:dbl, "Real output theta"=→"Real Output theta":dbl, "Step diff"=w960:dbl)  [unwired: 8 in]
            n181 = local write "Step difference L"(w960) -> ()
            n182 = local write "Step difference R"(w960) -> ()
          }
        }
        n183 = control-ref of="Motor Input L"() -> (w931:refnum<vi>)
        n184 = control-ref of="Motor Input R"() -> (w926:refnum<vi>)
        n185 = call "Single Axis motor_R(SubVI).vi"("State=1, I"=w922, "Motor=0, I"=w924, "Motor Input"="Motor Input R", "Step diff"="Step difference R", "Motor Input_L"=w926) -> ("right"=→"right R":bool, "State=1, O"=w921:dbl, "Motor=0, O"=w923:i32, "up"=w914:bool, "left"=w913:bool, "Moving"=→"Moving R":bool, "down"=→"down R":bool)  [unwired: 14 in, 2 out]
        "up R" <- w914
        "left R" <- w913
        n186 = call "Single Axis motor_L(SubVI).vi"("State=1, I"=w937, "Motor=0, I"=w935, "Motor Input"="Motor Input L", "Step diff"="Step difference L", "Motor Input_L"=w931) -> ("right"=→"right L":bool, "State=1, O"=w936:dbl, "Motor=0, O"=w934:i32, "up"=w908:bool, "left"=w907:bool, "Moving"=→"Moving":bool, "down"=→"down L":bool)  [unwired: 14 in, 2 out]
        "up L" <- w908
        "left L" <- w907
        n187 = local read "Stop"() -> (w929:bool)
        n188 = Build Array(w914) -> (w916:bool[])
        n189 = Build Array(w913) -> (w915:bool[])
        n190 = Reciprocal(x="Step/s  curve") -> (1/x=w945:dbl)
        n191 = Build Array(w908) -> (w910:bool[])
        n192 = Build Array(w907) -> (w909:bool[])
        n193 = call <vilib>:"Write.vi"("Values"=w916, "DIO Ref In"=w912) -> ("DIO Ref Out"=w902:T14)  [unwired: 7 in, 1 out]
        n194 = call <vilib>:"Write.vi"("Values"=w915, "DIO Ref In"=w911) -> ("DIO Ref Out"=w901:T14)  [unwired: 7 in, 1 out]
        n195 = Multiply(x=w945, y=1000) -> (x*y=w943:dbl)
        n196 = call <vilib>:"Write.vi"("Values"=w910, "DIO Ref In"=w905) -> ("DIO Ref Out"=w904:T14)  [unwired: 7 in, 1 out]
        n197 = call <vilib>:"Write.vi"("Values"=w909, "DIO Ref In"=w906) -> ("DIO Ref Out"=w903:T14)  [unwired: 7 in, 1 out]
        n198 = node-c288(w943) -> ()  [unwired: 1 out]
      }
      n199 = timed-loop {
        shift-right: [w800] -> w714
        shift-left: w722 -> [w811]
        shift-right: [w801] -> _
        shift-left: 1 -> [w812]
        shift-right: [w797] -> _
        shift-left: -25 -> [w810]
        timing: w735 -> [_]
        timing-out: [_] -> w734
        tunnel: w706 -> [w787]
        tunnel: w705 -> [w786]
        tunnel: [w785] -> w692
        tunnel: [w784] -> w691
        stop <- w795 stop-if-true
        n200 = node-c288() -> ()  [unwired: 1 in, 1 out]
        n201 = control-ref of="Motor Input y"() -> (w804:refnum<vi>)
        n202 = control-ref of="User Input y"() -> (w803:refnum<vi>)
        n203 = control-ref of="Step diff y"() -> (w802:refnum<vi>)
        n204 = local read "Stop"() -> (w795:bool)
        n205 = call "Single Axis motor_Y(SubVI).vi"("State=1, I"=w812, "Motor=0, I"=w811, "Position=0, I"=w810, "User Input"="User Input y", "Motor Input"="Motor Input y", "Backward"="Left y", "Forward"="Right y", "Step diff"="Step diff y", "Motor input_L"=w804, "User input_L"=w803, "Step diff_L"=w802) -> ("right"=→"right y":bool, "down"=→"down y":bool, "Motor State"=→"Motor State y":dbl, "State=1, O"=w801:dbl, "Motor=0, O"=w800:i32, "Position=0, O"=w797:dbl, "Real Output"=→"Real Output y":dbl, "Motor Position"=→"Motor Position y":dbl, "up"=w789:bool, "left"=w788:bool, "Moving"=→"Moving y":bool)  [unwired: 5 in, 1 out]
        "up y" <- w789
        "left y" <- w788
        n206 = Reciprocal(x="Step/s y") -> (1/x=w815:dbl)
        n207 = Build Array(w789) -> (w791:bool[])
        n208 = Build Array(w788) -> (w790:bool[])
        n209 = call <vilib>:"Write.vi"("Values"=w791, "DIO Ref In"=w787) -> ("DIO Ref Out"=w784:T14)  [unwired: 7 in, 1 out]
        n210 = call <vilib>:"Write.vi"("Values"=w790, "DIO Ref In"=w786) -> ("DIO Ref Out"=w785:T14)  [unwired: 7 in, 1 out]
        n211 = Multiply(x=w815, y=1000) -> (x*y=w813:dbl)
        n212 = node-c288(w813) -> ()  [unwired: 1 out]
      }
      n213 = timed-loop {
        shift-right: [w761] -> w712
        shift-left: w719 -> [w772]
        shift-right: [w762] -> _
        shift-left: 1 -> [w773]
        shift-right: [w757] -> _
        shift-left: 0 -> [w771]
        timing: w727 -> [_]
        timing-out: [_] -> w726
        tunnel: w708 -> [w748]
        tunnel: w707 -> [w747]
        tunnel: [w746] -> w688
        tunnel: [w745] -> w687
        stop <- w755 stop-if-true
        n214 = node-c288() -> ()  [unwired: 1 in, 1 out]
        n215 = control-ref of="Motor Input psi"() -> (w765:refnum<vi>)
        n216 = control-ref of="User Input psi"() -> (w764:refnum<vi>)
        n217 = control-ref of="Step diff psi"() -> (w763:refnum<vi>)
        n218 = local read "Stop"() -> (w755:bool)
        n219 = call "Single Axis motor_Psi(SubVI).vi"("State=1, I"=w773, "Motor=0, I"=w772, "Position=0, I"=w771, "User Input"="User Input psi", "Motor Input"="Motor Input psi", "Backward"="Left psi", "Forward"="Right psi", "Step diff"="Step diff psi", "Motor input_L"=w765, "User input_L"=w764, "Step diff_L"=w763) -> ("right"=→"right psi":bool, "down"=→"down psi":bool, "Motor State"=→"Motor State psi":dbl, "State=1, O"=w762:dbl, "Motor=0, O"=w761:i32, "Position=0, O"=w757:dbl, "Real Output"=→"Real Output psi":dbl, "Motor Position"=→"Motor Position psi":dbl, "up"=w750:bool, "left"=w749:bool, "Moving"=→"Moving psi":bool)  [unwired: 5 in, 1 out]
        "up psi" <- w750
        "left psi" <- w749
        n220 = Reciprocal(x="Step/s psi") -> (1/x=w776:dbl)
        n221 = Build Array(w750) -> (w752:bool[])
        n222 = Build Array(w749) -> (w751:bool[])
        n223 = call <vilib>:"Write.vi"("Values"=w752, "DIO Ref In"=w748) -> ("DIO Ref Out"=w745:T14)  [unwired: 7 in, 1 out]
        n224 = call <vilib>:"Write.vi"("Values"=w751, "DIO Ref In"=w747) -> ("DIO Ref Out"=w746:T14)  [unwired: 7 in, 1 out]
        n225 = Multiply(x=w776, y=1000) -> (x*y=w774:dbl)
        n226 = node-c288(w774) -> ()  [unwired: 1 out]
      }
      n227 = timed-loop {
        shift-right: [w880] -> w713
        shift-left: w721 -> [w889]
        shift-right: [w881] -> _
        shift-left: 1 -> [w890]
        shift-right: [w876] -> _
        shift-left: 25 -> [w888]
        timing: w739 -> [_]
        timing-out: [_] -> w738
        tunnel: w710 -> [w865]
        tunnel: w709 -> [w864]
        tunnel: [w863] -> w690
        tunnel: [w862] -> w689
        stop <- w874 stop-if-true
        n228 = node-c288() -> ()  [unwired: 1 in, 1 out]
        n229 = control-ref of="Motor Input z"() -> (w884:refnum<vi>)
        n230 = control-ref of="User Input z"() -> (w883:refnum<vi>)
        n231 = control-ref of="Step diff z"() -> (w882:refnum<vi>)
        n232 = call "Single Axis motor_Z(SubVI).vi"("State=1, I"=w890, "Motor=0, I"=w889, "Position=0, I"=w888, "User Input"="User Input z", "Motor Input"="Motor Input z", "Backward"="Down z", "Forward"="Up z", "Step diff"="Step diff z", "Motor input_L"=w884, "User input_L"=w883, "Step diff_L"=w882) -> ("right"=→"right z":bool, "down"=→"down z":bool, "Motor State"=→"Motor State z":dbl, "State=1, O"=w881:dbl, "Motor=0, O"=w880:i32, "Position=0, O"=w876:dbl, "Real Output"=→"Real Output z":dbl, "Motor Position"=→"Motor Position z":dbl, "up"=w866:bool, "left"=w867:bool, "Moving"=→"Moving z":bool)  [unwired: 5 in, 1 out]
        "up z" <- w866
        "left z" <- w867
        n233 = local read "Stop"() -> (w874:bool)
        n234 = Reciprocal(x="Step/s z") -> (1/x=w893:dbl)
        n235 = Build Array(w866) -> (w869:bool[])
        n236 = Build Array(w867) -> (w868:bool[])
        n237 = call <vilib>:"Write.vi"("Values"=w869, "DIO Ref In"=w865) -> ("DIO Ref Out"=w862:T14)  [unwired: 7 in, 1 out]
        n238 = call <vilib>:"Write.vi"("Values"=w868, "DIO Ref In"=w864) -> ("DIO Ref Out"=w863:T14)  [unwired: 7 in, 1 out]
        n239 = Multiply(x=w893, y=1000) -> (x*y=w891:dbl)
        n240 = node-c288(w891) -> ()  [unwired: 1 out]
      }
      n241 = node-c288(w743) -> ()  [unwired: 1 out]
      n242 = node-c288(w736) -> ()  [unwired: 1 out]
      n243 = node-c288(w734) -> ()  [unwired: 1 out]
      n244 = node-c288(w726) -> ()  [unwired: 1 out]
      n245 = node-c288(w738) -> ()  [unwired: 1 out]
    }
    frame #4 {
      n246 = node-c288() -> (w999:T3)  [unwired: 4 in]
      n247 = node-c288() -> (w1002:T3)  [unwired: 4 in]
      n248 = node-c288() -> (w1005:T3)  [unwired: 4 in]
      n249 = node-c288() -> (w1008:T3)  [unwired: 4 in]
      n250 = node-c288() -> (w1011:T3)  [unwired: 4 in]
      n251 = node-c288() -> (w1014:T3)  [unwired: 4 in]
      n252 = timed-loop {
        timing: w999 -> [_]
        timing-out: [_] -> w998
        shift-right: [w1024] -> _
        shift-left: w997 -> [w1028]
        tunnel: w997 -> [w1029]
        tunnel: w980 -> [w1018]
        tunnel: w979 -> [w1017]
        tunnel: [w1016] -> w974
        tunnel: [w1015] -> w973
        i -> [w1027]
        stop <- w1023 stop-if-true
        n253 = node-c288() -> ()  [unwired: 1 in, 1 out]
        n254 = control-ref of="Stop number psi"() -> (w1025:refnum<vi>)
        n255 = call "Motor stop_Psi(SubVI).vi"("Motor, C"=w1029, "Motor, I"=w1028, "i"=w1027, "Stop number"="Stop number psi", "Stop number_L"=w1025) -> ("Motor, O"=w1024:i32, "Loop stop"=w1023:bool, "up"=w1020:bool, "left"=w1019:bool)  [unwired: 7 in]
        n256 = Build Array(w1020) -> (w1021:bool[])
        n257 = Build Array(w1019) -> (w1022:bool[])
        n258 = call <vilib>:"Write.vi"("Values"=w1021, "DIO Ref In"=w1017) -> ("DIO Ref Out"=w1016:T14)  [unwired: 7 in, 1 out]
        n259 = call <vilib>:"Write.vi"("Values"=w1022, "DIO Ref In"=w1018) -> ("DIO Ref Out"=w1015:T14)  [unwired: 7 in, 1 out]
        n260 = node-c288(100) -> ()  [unwired: 1 out]
      }
      n261 = timed-loop {
        timing: w1002 -> [_]
        timing-out: [_] -> w1001
        shift-right: [w1046] -> _
        shift-left: w1000 -> [w1050]
        tunnel: w1000 -> [w1051]
        tunnel: w982 -> [w1039]
        tunnel: w981 -> [w1040]
        tunnel: [w1038] -> w976
        tunnel: [w1037] -> w975
        i -> [w1049]
        stop <- w1045 stop-if-true
        n262 = node-c288() -> ()  [unwired: 1 in, 1 out]
        n263 = control-ref of="Stop number z"() -> (w1047:refnum<vi>)
        n264 = call "Motor stop_Z(SubVI).vi"("Motor, C"=w1051, "Motor, I"=w1050, "i"=w1049, "Stop number"="Stop number z", "Stop number_L"=w1047) -> ("Motor, O"=w1046:i32, "Loop stop"=w1045:bool, "up"=w1042:bool, "left"=w1041:bool)  [unwired: 7 in]
        n265 = Build Array(w1042) -> (w1043:bool[])
        n266 = Build Array(w1041) -> (w1044:bool[])
        n267 = call <vilib>:"Write.vi"("Values"=w1043, "DIO Ref In"=w1040) -> ("DIO Ref Out"=w1038:T14)  [unwired: 7 in, 1 out]
        n268 = call <vilib>:"Write.vi"("Values"=w1044, "DIO Ref In"=w1039) -> ("DIO Ref Out"=w1037:T14)  [unwired: 7 in, 1 out]
        n269 = node-c288(100) -> ()  [unwired: 1 out]
      }
      n270 = timed-loop {
        timing: w1005 -> [_]
        timing-out: [_] -> w1004
        shift-right: [w1068] -> _
        shift-left: w1003 -> [w1072]
        tunnel: w1003 -> [w1073]
        tunnel: w984 -> [w1062]
        tunnel: w983 -> [w1061]
        tunnel: [w1060] -> w978
        tunnel: [w1059] -> w977
        i -> [w1071]
        stop <- w1067 stop-if-true
        n271 = node-c288() -> ()  [unwired: 1 in, 1 out]
        n272 = control-ref of="Stop number y"() -> (w1069:refnum<vi>)
        n273 = call "Motor stop_Y(SubVI).vi"("Motor, C"=w1073, "Motor, I"=w1072, "i"=w1071, "Stop number"="Stop number y", "Stop number_L"=w1069) -> ("Motor, O"=w1068:i32, "Loop stop"=w1067:bool, "up"=w1064:bool, "left"=w1063:bool)  [unwired: 7 in]
        n274 = Build Array(w1064) -> (w1065:bool[])
        n275 = Build Array(w1063) -> (w1066:bool[])
        n276 = call <vilib>:"Write.vi"("Values"=w1065, "DIO Ref In"=w1061) -> ("DIO Ref Out"=w1060:T14)  [unwired: 7 in, 1 out]
        n277 = call <vilib>:"Write.vi"("Values"=w1066, "DIO Ref In"=w1062) -> ("DIO Ref Out"=w1059:T14)  [unwired: 7 in, 1 out]
        n278 = node-c288(100) -> ()  [unwired: 1 out]
      }
      n279 = timed-loop {
        timing: w1008 -> [_]
        timing-out: [_] -> w1007
        shift-right: [w1090] -> _
        shift-left: w1006 -> [w1094]
        tunnel: w1006 -> [w1095]
        tunnel: [w1084] -> w988
        tunnel: [w1083] -> w987
        tunnel: w986 -> [w1082]
        tunnel: w985 -> [w1081]
        i -> [w1093]
        stop <- w1089 stop-if-true
        n280 = node-c288() -> ()  [unwired: 1 in, 1 out]
        n281 = control-ref of="Stop number x"() -> (w1091:refnum<vi>)
        n282 = call "Motor stop_X(SubVI).vi"("Motor, C"=w1095, "Motor, I"=w1094, "i"=w1093, "Stop number"="Stop number x", "Stop number_L"=w1091) -> ("Motor, O"=w1090:i32, "Loop stop"=w1089:bool, "up"=w1086:bool, "left"=w1085:bool)  [unwired: 7 in]
        n283 = Build Array(w1086) -> (w1087:bool[])
        n284 = Build Array(w1085) -> (w1088:bool[])
        n285 = call <vilib>:"Write.vi"("Values"=w1087, "DIO Ref In"=w1081) -> ("DIO Ref Out"=w1084:T14)  [unwired: 7 in, 1 out]
        n286 = call <vilib>:"Write.vi"("Values"=w1088, "DIO Ref In"=w1082) -> ("DIO Ref Out"=w1083:T14)  [unwired: 7 in, 1 out]
        n287 = node-c288(100) -> ()  [unwired: 1 out]
      }
      n288 = timed-loop {
        timing: w1011 -> [_]
        timing-out: [_] -> w1010
        shift-right: [w1112] -> _
        shift-left: w1009 -> [w1116]
        tunnel: w1009 -> [w1117]
        tunnel: w992 -> [w1106]
        tunnel: w991 -> [w1105]
        tunnel: [w1104] -> w990
        tunnel: [w1103] -> w989
        i -> [w1115]
        stop <- w1111 stop-if-true
        n289 = node-c288() -> ()  [unwired: 1 in, 1 out]
        n290 = control-ref of="Stop number R"() -> (w1113:refnum<vi>)
        n291 = call "Motor stop_R(SubVI).vi"("Motor, C"=w1117, "Motor, I"=w1116, "i"=w1115, "Stop number"="Stop number R", "Stop number_L"=w1113) -> ("Motor, O"=w1112:i32, "Loop stop"=w1111:bool, "up"=w1108:bool, "left"=w1107:bool)  [unwired: 7 in]
        n292 = Build Array(w1108) -> (w1109:bool[])
        n293 = Build Array(w1107) -> (w1110:bool[])
        n294 = call <vilib>:"Write.vi"("Values"=w1109, "DIO Ref In"=w1106) -> ("DIO Ref Out"=w1104:T14)  [unwired: 7 in, 1 out]
        n295 = call <vilib>:"Write.vi"("Values"=w1110, "DIO Ref In"=w1105) -> ("DIO Ref Out"=w1103:T14)  [unwired: 7 in, 1 out]
        n296 = node-c288(100) -> ()  [unwired: 1 out]
      }
      n297 = timed-loop {
        timing: w1014 -> [_]
        timing-out: [_] -> w1013
        shift-right: [w1134] -> _
        shift-left: w1012 -> [w1138]
        tunnel: w1012 -> [w1139]
        tunnel: [w1128] -> w996
        tunnel: [w1127] -> w995
        tunnel: w994 -> [w1126]
        tunnel: w993 -> [w1125]
        i -> [w1137]
        stop <- w1133 stop-if-true
        n298 = node-c288() -> ()  [unwired: 1 in, 1 out]
        n299 = control-ref of="Stop number L"() -> (w1135:refnum<vi>)
        n300 = call "Motor stop_L(SubVI).vi"("Motor, C"=w1139, "Motor, I"=w1138, "i"=w1137, "Stop number"="Stop number L", "Stop number_L"=w1135) -> ("Motor, O"=w1134:i32, "Loop stop"=w1133:bool, "up"=w1130:bool, "left"=w1129:bool)  [unwired: 7 in]
        n301 = Build Array(w1130) -> (w1131:bool[])
        n302 = Build Array(w1129) -> (w1132:bool[])
        n303 = call <vilib>:"Write.vi"("Values"=w1131, "DIO Ref In"=w1126) -> ("DIO Ref Out"=w1128:T14)  [unwired: 7 in, 1 out]
        n304 = call <vilib>:"Write.vi"("Values"=w1132, "DIO Ref In"=w1125) -> ("DIO Ref Out"=w1127:T14)  [unwired: 7 in, 1 out]
        n305 = node-c288(100) -> ()  [unwired: 1 out]
      }
      n306 = node-c288(w998) -> ()  [unwired: 1 out]
      n307 = node-c288(w1001) -> ()  [unwired: 1 out]
      n308 = node-c288(w1004) -> ()  [unwired: 1 out]
      n309 = call <vilib>:"Close.vi"("DIO Ref In"=w974) -> ()  [unwired: 10 in, 1 out]
      n310 = call <vilib>:"Close.vi"("DIO Ref In"=w973) -> ()  [unwired: 10 in, 1 out]
      n311 = node-c288(w1007) -> ()  [unwired: 1 out]
      n312 = call <vilib>:"Close.vi"("DIO Ref In"=w976) -> ()  [unwired: 10 in, 1 out]
      n313 = call <vilib>:"Close.vi"("DIO Ref In"=w975) -> ()  [unwired: 10 in, 1 out]
      n314 = node-c288(w1010) -> ()  [unwired: 1 out]
      n315 = call <vilib>:"Close.vi"("DIO Ref In"=w978) -> ()  [unwired: 10 in, 1 out]
      n316 = node-c288(w1013) -> ()  [unwired: 1 out]
      n317 = call <vilib>:"Close.vi"("DIO Ref In"=w977) -> ()  [unwired: 10 in, 1 out]
      n318 = call <vilib>:"Close.vi"("DIO Ref In"=w988) -> ()  [unwired: 10 in, 1 out]
      n319 = call <vilib>:"Close.vi"("DIO Ref In"=w987) -> ()  [unwired: 10 in, 1 out]
      n320 = call <vilib>:"Close.vi"("DIO Ref In"=w996) -> ()  [unwired: 10 in, 1 out]
      n321 = call <vilib>:"Close.vi"("DIO Ref In"=w995) -> ()  [unwired: 10 in, 1 out]
      n322 = call <vilib>:"Close.vi"("DIO Ref In"=w990) -> ()  [unwired: 10 in, 1 out]
      n323 = call <vilib>:"Close.vi"("DIO Ref In"=w989) -> ()  [unwired: 10 in, 1 out]
    }
  }
